vi "DMM Read Diode Voltage.vi"(0 "instrument handle":refnum<k15>, 11 "error in":errorcluster) -> (4 "instrument handle out":refnum<k15>, 6 "Diode Voltage (V)":dbl, 8 "Over Range?":bool, 15 "error out":errorcluster)   [LabVIEW 2026]
doc: "Configures the NI-DMM session for the Diode function (1 mA source) on the 10 V range with 6.5 digits, takes 5 readings and returns their mean as Diode Voltage. A WARNING from the driver (for example over-range on an open or regulated cell) is cleared and reported as Over Range? TRUE instead of being passed on; Over Range? is also TRUE when the mean is 4.0 V or more or not a number. A real error passes through. Leaves the DMM in diode mode and does not open or close the session."
uses:
  <vilib>/Analysis/NI_AALBase.lvlib
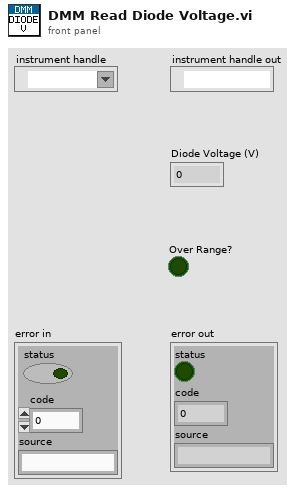
[diagram p1: front panel]
types:
  T1 = enum16{"Immediate", "External", "TTL 0", "TTL 1", "TTL 2", "TTL 3", "TTL 4", "TTL 5", "TTL 6", "Interval", "Software", "TTL 7", "PXI Star", "LBR Trig 1", "Aux Trig 1"}
  T2 = enum16{"DC Volts", "AC Volts", "DC Current", "AC Current", "2-wire Resistance", "4-wire Resistance", "Diode", "Frequency", "Period", "AC Volts DC Coupled", "Capacitance", "Inductance", "Temperature"}
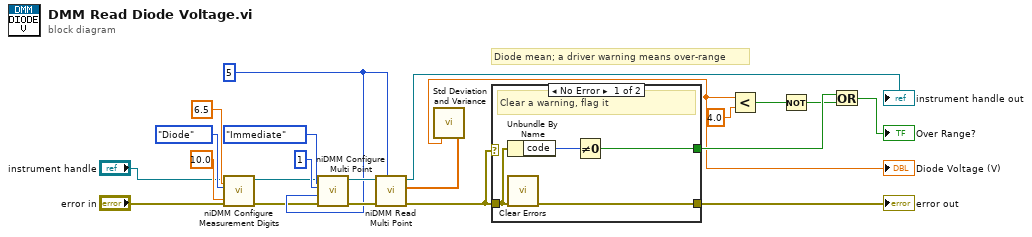
[diagram p0: block diagram]
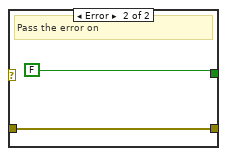
[diagram p2: hidden frame]
diagram:
  w9 = 5 ("Number to Read")
  # "Diode mean; a driver warning means over-range"
  n1 = call <instrlib>:"niDMM Configure Measurement Digits.vi"("Range"=10.0, "Resolution in Digits"=6.5, "error in (no error)"="error in", "Function"=T2."Diode", "instrument handle"="instrument handle") -> ("error out"=w6:errorcluster, "instrument handle out"=w7:refnum<k15>)  [unwired: 5 in]
  n2 = call <instrlib>:"niDMM Configure Multi Point.vi"("Sample Trigger"=T1."Immediate", "error in (no error)"=w6, "Sample Count"=w9, "Trigger Count"=1, "instrument handle"=w7) -> ("error out"=w11:errorcluster, "instrument handle out"=w12:refnum<k15>)  [unwired: 5 in]
  n3 = call <instrlib>:"niDMM Read Multi Point.vi"("Number to Read"=w9, "error in (no error)"=w11, "instrument handle"=w12) -> ("error out"=w13:errorcluster, "Measurements"=w14:dbl[], "instrument handle out"=→"instrument handle out":refnum<k15>)  [unwired: 5 in, 1 out]
  n4 = call <vilib>:"Std Deviation and Variance.vi"("X"=w14) -> ("mean"=w16:dbl)  [unwired: 1 in, 2 out]
  "Diode Voltage (V)" <- w16
  n5 = case shown="No Error" w13 {
    tunnel: w13 -> [w23 w27]
    tunnel: [w26 w27] -> w20
    tunnel: [w25 FALSE ("no warning")] -> w21
    frame No Error {
      # "Clear a warning, flag it"
      n6 = Unbundle By Name(w23) -> ("code"=w24:i32)
      n7 = call <vilib>:"Clear Errors.vi"("error in (no error)"=w23) -> ("error out"=w26:errorcluster)  [unwired: 5 in, 1 out]
      n8 = Not Equal To 0?(x=w24) -> (x != 0?=w25:bool)
    }
    frame Error {
      # "Pass the error on"
    }
  }
  "error out" <- w20
  n9 = Less?(x=w16, y=4.0 ("clamp limit")) -> (x < y?=w18:bool)
  n10 = Not(x=w18) -> (.not. x?=w19:bool)
  n11 = Or(x=w21, y=w19) -> (x .or. y?=→"Over Range?":bool)
